vi "Init WS Manager.vi"(8 "error in (no error)":errorcluster, 11 "Basic WebSocket Manager in":refnum<class "Basic WebSocket Manager.lvclass">) -> (0 "error out":errorcluster, 3 "Basic WebSocket Manager out":refnum<class "Basic WebSocket Manager.lvclass">)   [LabVIEW 2020, in "HTTP Server.lvlib" / "Basic WebSocket Manager.lvclass"]
uses:
  Basic WebSocket Manager.lvclass
  Ref Data.ctl
  WebSocket Client/WebSocket Client.lvclass
  Basic WebSocket Manager.lvclass/Basic WebSocket Manager.ctl
  WebSocket Format.ctl
  HTTP Server.lvlib
  WS Payload.ctl
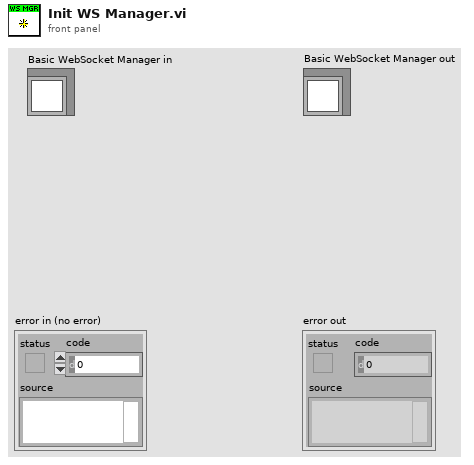
[diagram p1: front panel]
types:
  T1 = typedef "HTTP Server.lvlib/Basic WebSocket Manager.lvclass/WS Payload.ctl" = cluster{"Format":T2, "Payload":string}
  T2 = typedef "HTTP Server.lvlib/WebSocket Format.ctl" = enum16{"Text", "Binary"}
  T3 = typedef "HTTP Server.lvlib/Basic WebSocket Manager.lvclass/Ref Data.ctl" = cluster{"Clients":map{string, refnum<class "WebSocket Client.lvclass">}}
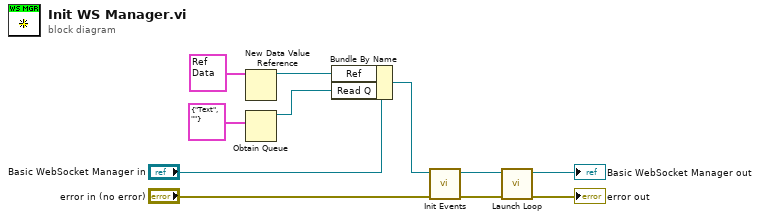
[diagram p0: block diagram]
diagram:
  n1 = New Data Value Reference(data value=T3 {"Clients"={}} ("Ref Data")) -> (data value reference=w8:refnum<data-value>)  [unwired: 1 in, 1 out]
  n2 = Obtain Queue(element data type=T1 {"Format"=enum."Text", "Payload"=""} ("WS Payload")) -> (queue out=w1:refnum<queue>)  [unwired: 4 in, 2 out]
  n3 = Bundle By Name(cluster="Basic WebSocket Manager in", "Ref"=w8, "Read Q"=w1) -> (w6:refnum<class "Basic WebSocket Manager.lvclass">)
  n4 = call "Init Events.vi"("error in (no error)"="error in (no error)", "Basic WebSocket Manager in"=w6) -> ("error out"=w7:errorcluster, "Basic WebSocket Manager out"=w4:refnum<class "Basic WebSocket Manager.lvclass">)  [unwired: 8 in]
  n5 = call "Launch Loop.vi"("error in (no error)"=w7, "Basic WebSocket Manager in"=w4) -> ("error out"=→"error out":errorcluster, "Basic WebSocket Manager out"=→"Basic WebSocket Manager out":refnum<class "Basic WebSocket Manager.lvclass">)  [unwired: 8 in]
